vi "J1939 Host Automation API_Example.vi"() -> ()   [LabVIEW 2019]
panel:
  out "error out":errorcluster
  out "Found DTCs":i32=6
  out "Status":enum16{"NOT_PRESENT", "ACTIVE", "INACTIVE"}(ring)
  in  "Expected DTC":string="75301.07"
  in  "Address":string="249"
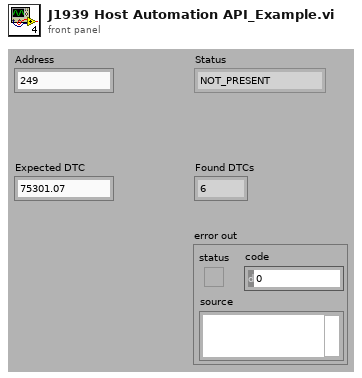
[diagram p1: front panel]
types:
  T1 = typedef "Host Automation API.lvlibp/NI STM.lvlib/TCP Connection Info.ctl" = cluster{"connection ID":refnum<k5>, "meta data":T2[]}
  T2 = typedef "Host Automation API.lvlibp/NI STM.lvlib/MetaDataElement.ctl" = string
  T3 = typedef "Host Automation API.lvlibp/Verify DTC_Status.ctl" = enum16{"NOT_PRESENT", "ACTIVE", "INACTIVE"}
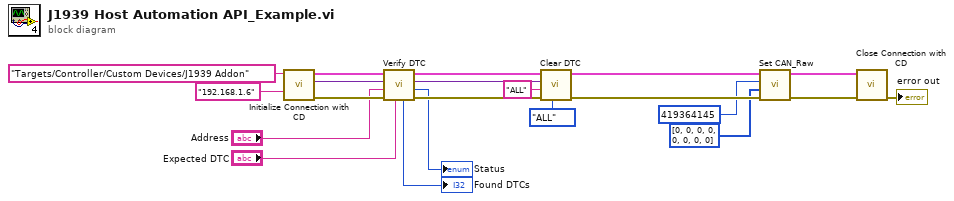
[diagram p0: block diagram]
diagram:
  n1 = call "Initialize Connection with CD.vi"("Unit Computer Address"="192.168.1.6", "Custom Device Path"="Targets/Controller/Custom Devices/J1939 Addon") -> ("error out"=w17:errorcluster, "Address Lookup Table"=w16:variant, "connection info"=w21:T1)  [unwired: 7 in]
  n2 = call "Verify DTC.vi"("Expected DTC"="Expected DTC", "error in"=w17, "Address"="Address", "Address Lookup Table"=w16, "connection info"=w21) -> ("error out"=w19:errorcluster, "Status"=→"Status":T3, "Address Lookup Table Out"=w18:variant, "connection info"=w20:T1, "Found DTCs"=→"Found DTCs":i32)  [unwired: 2 in]
  n3 = call "Clear DTC.vi"("Action"=enum16{"ALL", "ACTIVE", "INACTIVE"}."ALL", "error in"=w19, "Address (ALL)"="ALL" ("TLA (ALL)"), "Address Lookup Table"=w18, "connection info"=w20) -> ("error out"=w6:errorcluster, "connection info"=w8:T1)  [unwired: 4 in, 1 out]
  n4 = call "Set CAN_Raw.vi"("error in (no error)"=w6, "Data"=u8[] [0, 0, 0, 0, 0, 0, 0, 0], "Identifier"=u32 419364145, "connection info"=w8) -> ("error out"=w5:errorcluster, "connection info"=w7:T1)  [unwired: 5 in, 1 out]
  n5 = call "Close Connection with CD.vi"("error in (no error)"=w5, "connection info"=w7) -> ("error out"=→"error out":errorcluster)  [unwired: 9 in]
